vi "NMR_Main.vi"() -> ()   [LabVIEW 2024]
uses:
  SpinCore_API_file_location.vi
  Serial Port.vi
  <vilib>/Instr/_visa.llb/VISA Configure Serial Port (Instr).vi
  GPIB_Address.vi
panel:
  in  "GPIB Address":string="23"
  in  "WindFreak resource name":refnum<visa-resource-name>="COM3"
  in  "XY8-1":bool
  in  "Spin Echo":bool
  in  "NV-T1":bool
  in  "NV-ESR":bool
  in  "Path to spinapi.dll":path=path "C:/SpinCore/SpinAPI/lib/spinapi64.dll"
  in  "Rabi":bool
  in  "Program Stop":bool
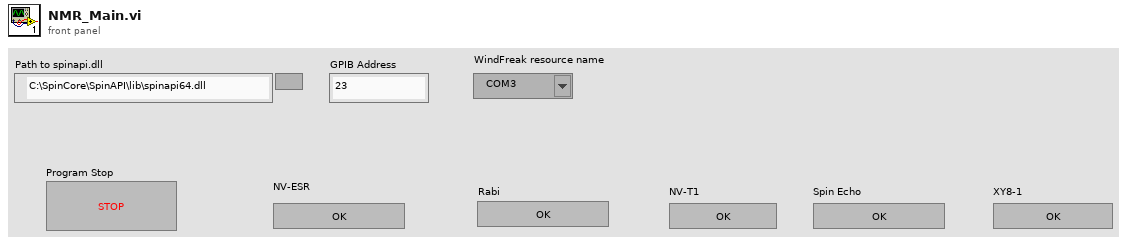
[diagram p1: front panel]
types:
  T1 = enum16{"Initialization", "Waiting for Input", "NV-ESR", "Rabi", "NV-T1", "Spin Echo", "XY8-1", "Exit"}
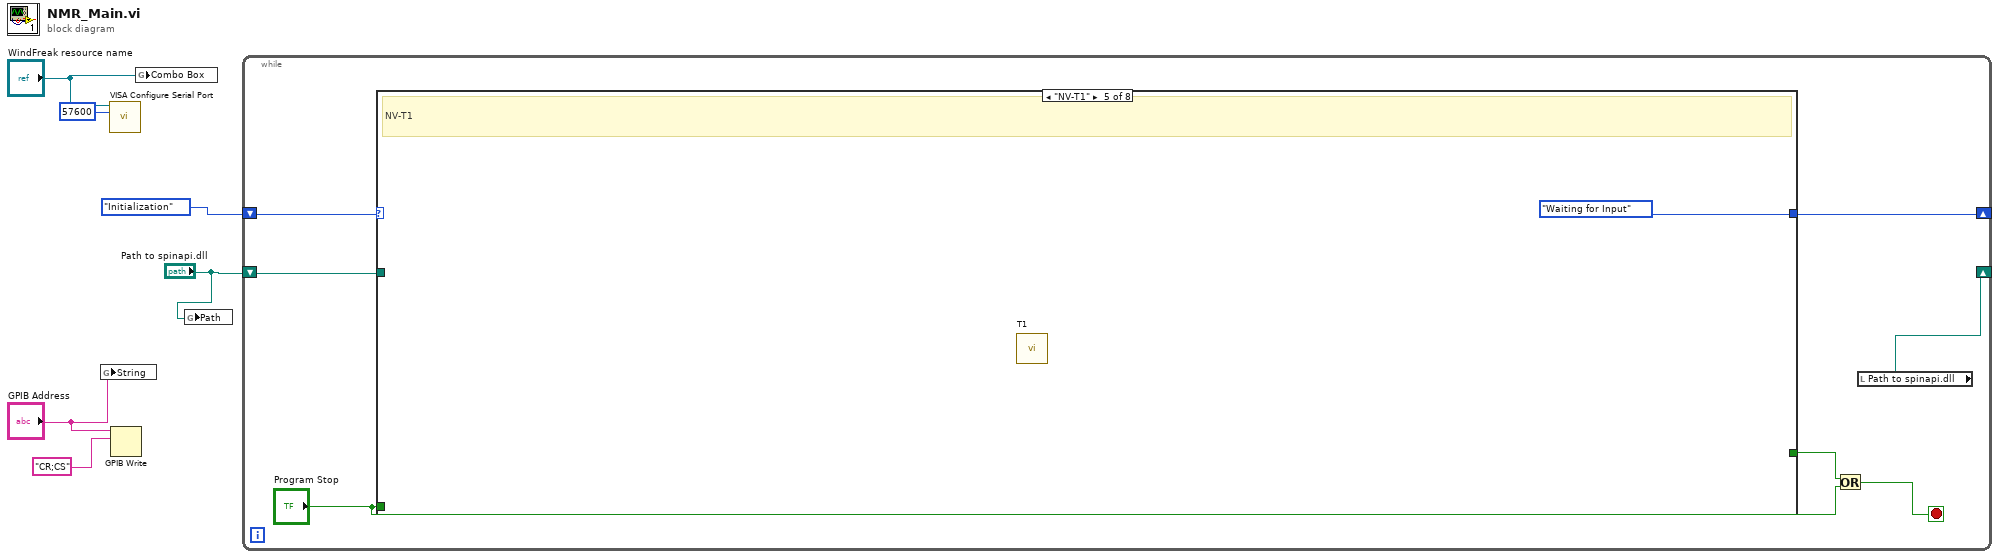
[diagram p0: block diagram]
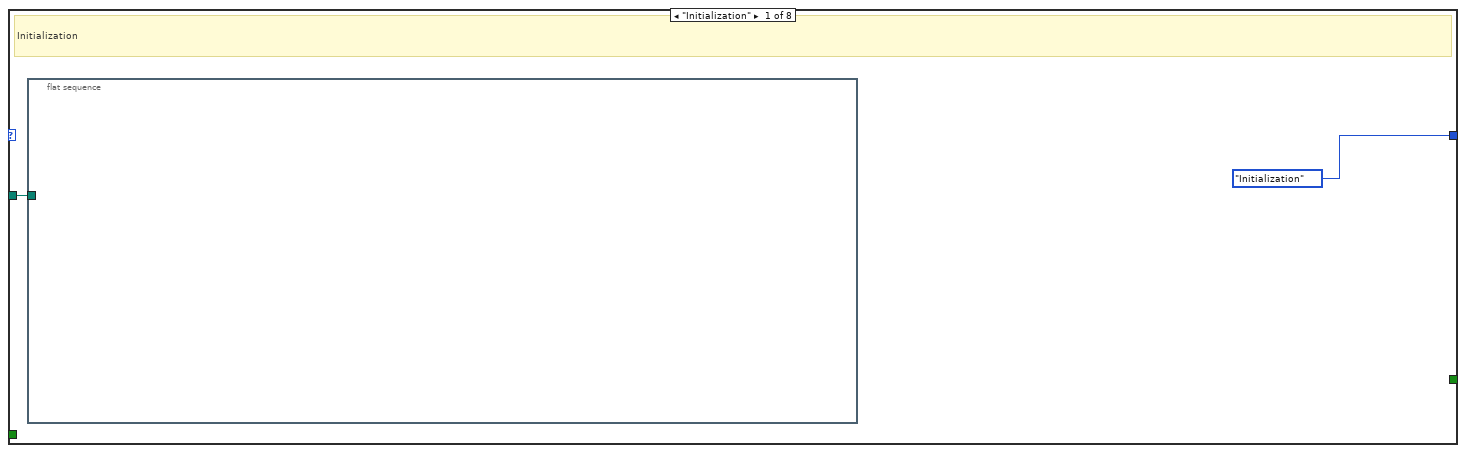
[diagram p2: hidden frame]
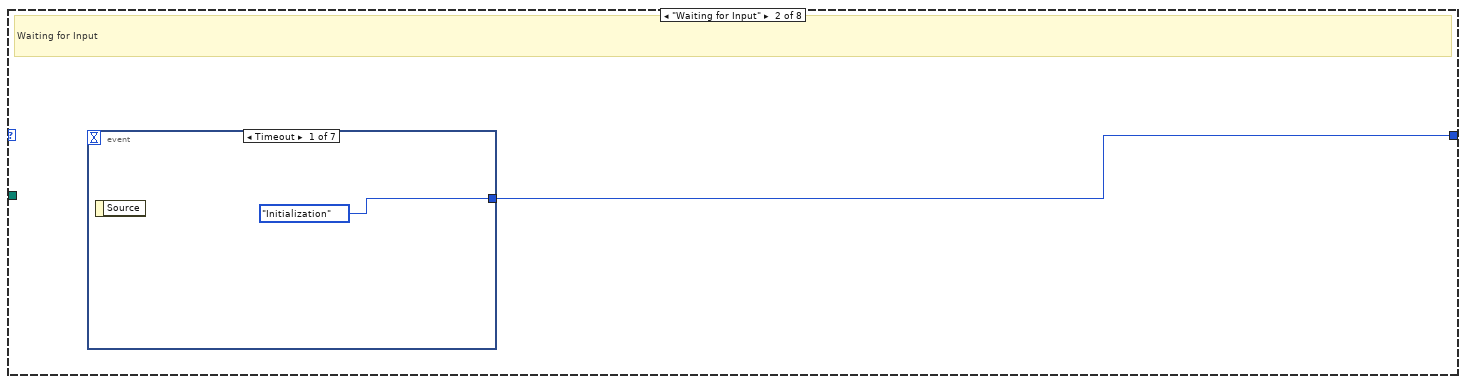
[diagram p3: hidden frame]
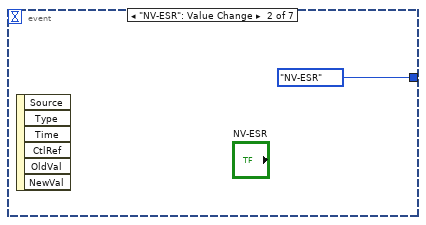
[diagram p4: hidden frame]
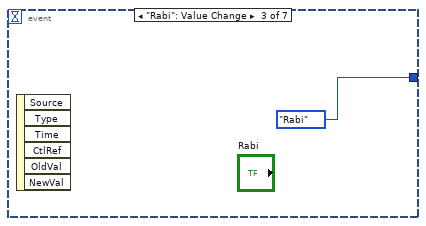
[diagram p5: hidden frame]
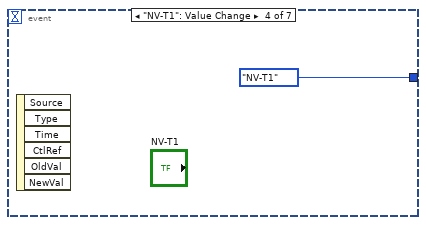
[diagram p6: hidden frame]
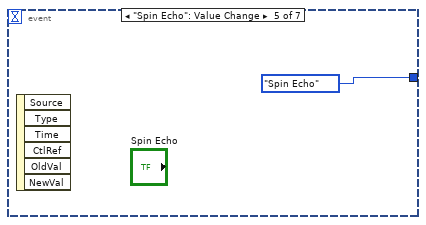
[diagram p7: hidden frame]
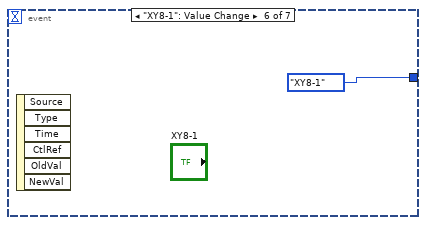
[diagram p8: hidden frame]
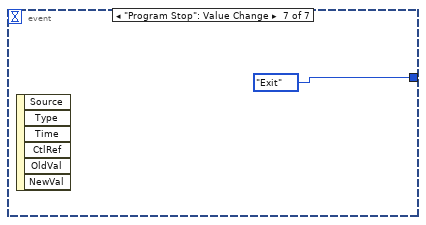
[diagram p9: hidden frame]
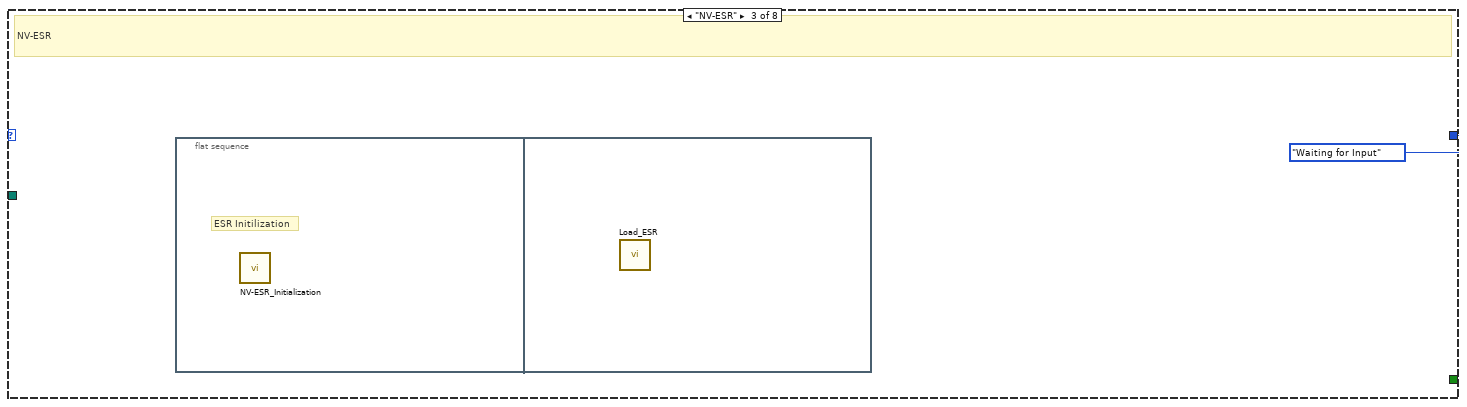
[diagram p10: hidden frame]
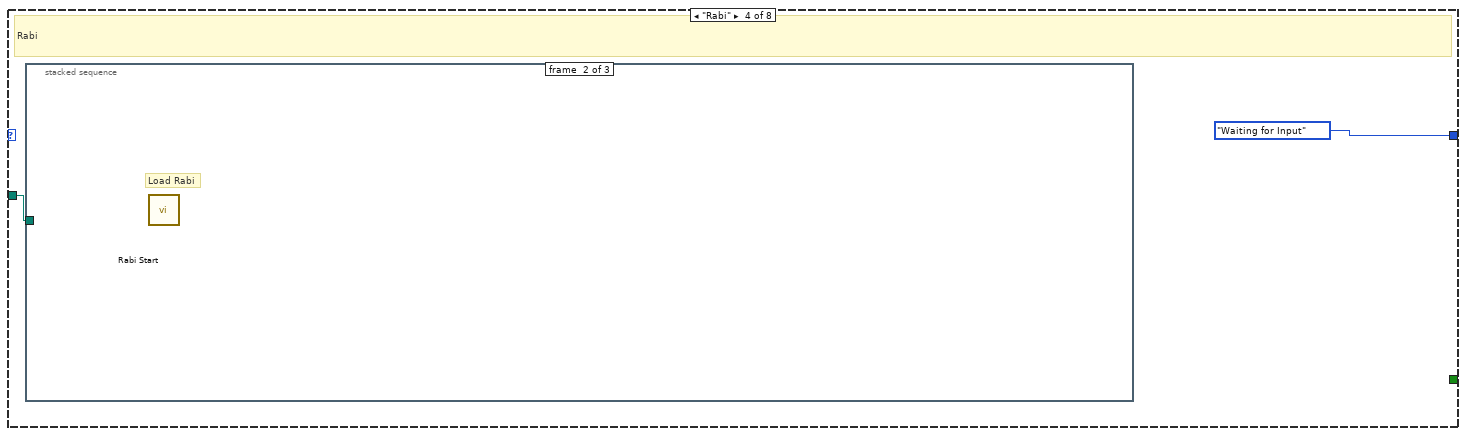
[diagram p11: hidden frame]
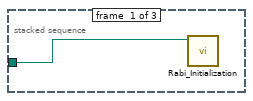
[diagram p12: hidden frame]
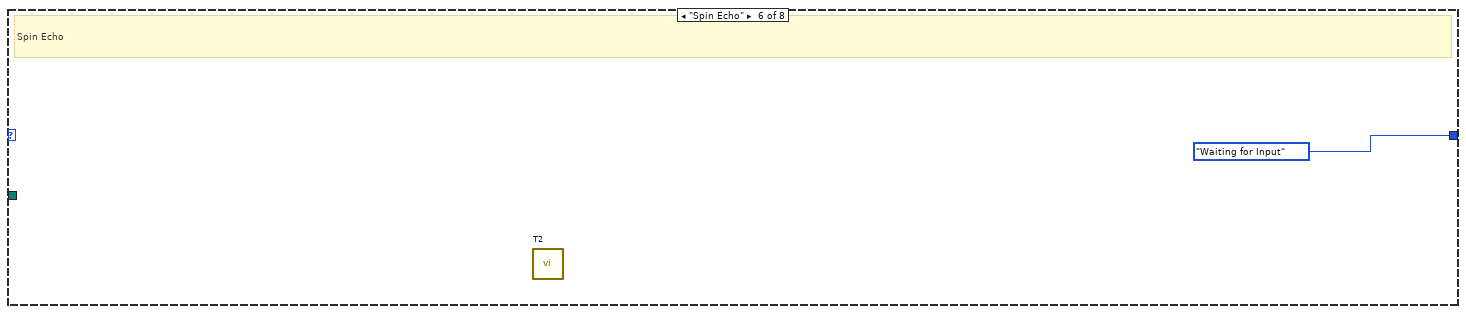
[diagram p14: hidden frame]
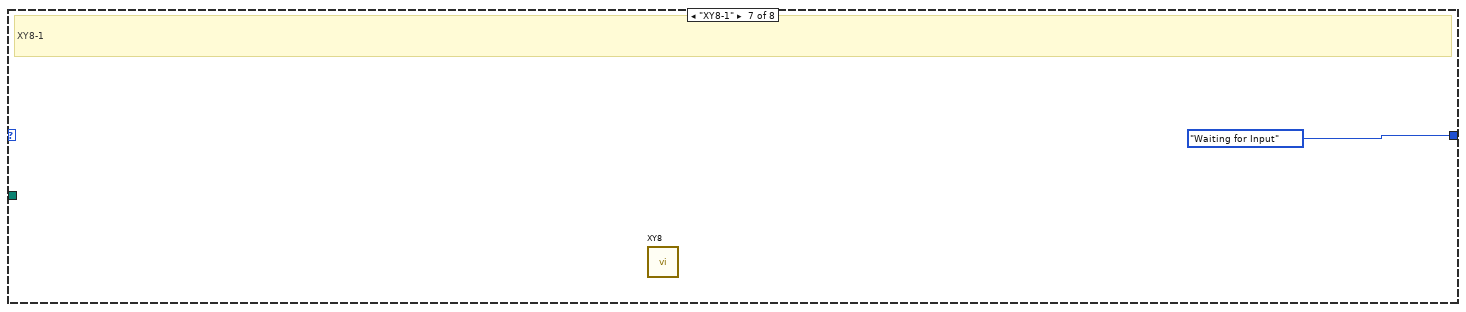
[diagram p15: hidden frame]
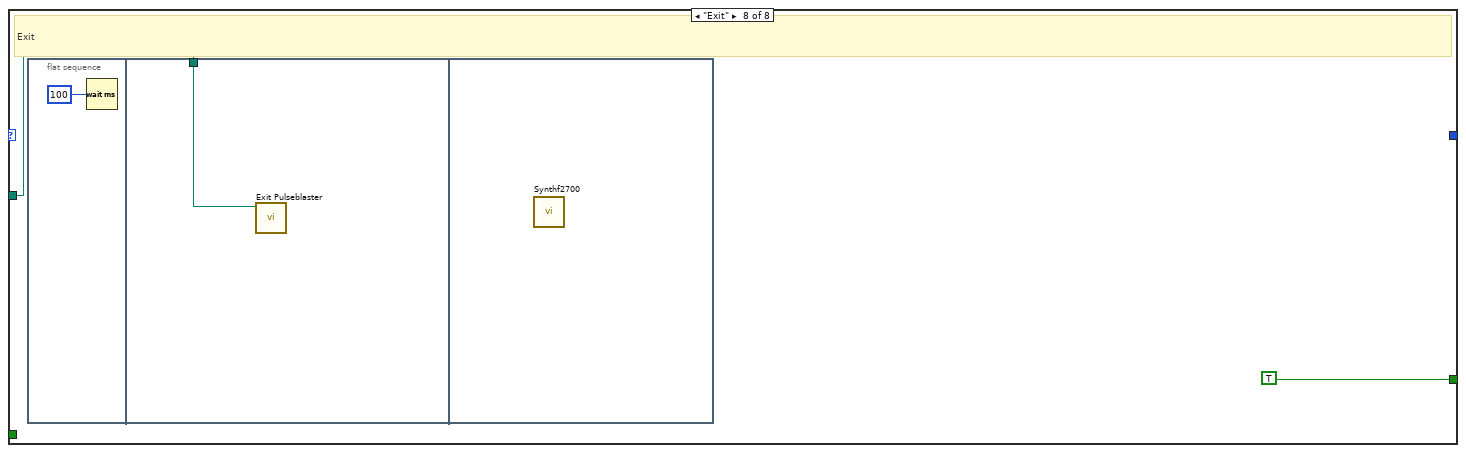
[diagram p16: hidden frame]
diagram:
  n1 = global write "GPIB_Address.vi" "String"("GPIB Address") -> ()
  n2 = call-poly "VISA Configure Serial Port"("VISA resource name"="WindFreak resource name", "baud rate (9600)"=u32 57600) -> ()  [unwired: 12 in, 2 out]
  n3 = GPIB Write(0:"GPIB Address", 1:"CR;CS" ("data")) -> ()  [unwired: 3 in, 2 out]
  n4 = global write "Serial Port.vi" "Combo Box"("WindFreak resource name") -> ()
  n5 = global write "SpinCore_API_file_location.vi" "Path"("Path to spinapi.dll") -> ()
  n6 = while {
    shift-right: [w13] -> _
    shift-left: T1."Initialization" -> [w12]
    shift-right: [w7] -> _
    shift-left: "Path to spinapi.dll" -> [w8]
    stop <- w9 stop-if-true
    n7 = case shown="\"NV-T1\"" w12 {
      tunnel: [T1."Initialization" w16 T1."Waiting for Input" T1."Waiting for Input" T1."Waiting for Input" T1."Waiting for Input" T1."Waiting for Input" _] -> w13
      tunnel: "Program Stop" -> [_ _ _ _ _ _ _ _]
      tunnel: [_ _ _ _ _ _ _ TRUE ("Program Stop")] -> w11
      tunnel: w8 -> [w15 _ _ w26 _ _ _ w31]
      frame "Initialization" {
        # "Initialization"
        n8 = flat-sequence {
          tunnel: w15 -> [_]
          frame #0 {
          }
        }
      }
      frame "Waiting for Input" {
        # "Waiting for Input"
        n9 = event shown="[0] Timeout" {
          selector: _ -> [_ _ _ _ _ _ _]
          dyn-events: _ -> [_ _ _ _ _ _ _]
          timeout: _ -> [_ _ _ _ _ _ _]
          tunnel: [T1."Initialization" T1."NV-ESR" T1."Rabi" T1."NV-T1" T1."Spin Echo" T1."XY8-1" T1."Exit"] -> w16
          event Timeout {
            n10 = event-data() -> ()  [unwired: 1 in, 1 out]
          }
          event "NV-ESR": Value Change {
            n11 = event-data() -> ()  [unwired: 1 in, 6 out]
          }
          event "Rabi": Value Change {
            n12 = event-data() -> ()  [unwired: 1 in, 6 out]
          }
          event "NV-T1": Value Change {
            n13 = event-data() -> ()  [unwired: 1 in, 6 out]
          }
          event "Spin Echo": Value Change {
            n14 = event-data() -> ()  [unwired: 1 in, 6 out]
          }
          event "XY8-1": Value Change {
            n15 = event-data() -> ()  [unwired: 1 in, 6 out]
          }
          event "Program Stop": Value Change {
            n16 = event-data() -> ()  [unwired: 1 in, 6 out]
          }
        }
      }
      frame "NV-ESR" {
        # "NV-ESR"
        n17 = flat-sequence {
          frame #0 {
            # "ESR Initilization"
            n18 = call "NV-ESR_Initialization.vi"() -> ()  [unwired: 12 in]
          }
          frame #1 {
            n19 = call "Load_ESR.vi"() -> ()  [unwired: 9 in, 3 out]
          }
        }
      }
      frame "Rabi" {
        # "Rabi"
        n20 = stacked-sequence {
          tunnel: w26 -> [w27 _ _]
          frame #0 {
            n21 = call "Rabi_Initialization.vi"("Path to spinapi.dll"=w27) -> ()  [unwired: 10 in, 1 out]
          }
          frame #1 {
            # "Load Rabi"
            n22 = call "Rabi Start.vi"() -> ()  [unwired: 12 in]
          }
          frame #2 {
          }
        }
      }
      frame "NV-T1" {
        # "NV-T1"
        n23 = call "T1.vi"() -> ()  [unwired: 12 in]
      }
      frame "Spin Echo" {
        # "Spin Echo"
        n24 = call "T2.vi"() -> ()  [unwired: 12 in]
      }
      frame "XY8-1" {
        # "XY8-1"
        n25 = call "XY8.vi"() -> ()  [unwired: 12 in]
      }
      frame "Exit" {
        # "Exit"
        n26 = flat-sequence {
          tunnel: w31 -> [w34]
          frame #0 {
            n27 = Wait (ms)(milliseconds to wait=u32 100) -> ()  [unwired: 1 out]
          }
          frame #1 {
            n28 = call "Exit Pulseblaster.vi"("Path to spinapi.dll"=w34) -> ()  [unwired: 11 in]
          }
          frame #2 {
            n29 = call "Synthf2700.vi"() -> ()  [unwired: 12 in]
          }
        }
      }
    }
    n30 = Or(x=w11, y="Program Stop") -> (x .or. y?=w9:bool)
    n31 = local read "Path to spinapi.dll"() -> (w7:path)
  }
